vi "Input&output.vi"() -> ()   [LabVIEW 2021]
uses:
  Option control.ctl
panel:
  in  "Tab Control":enum32{"Page 2"}(tab)
  in  "LOG ID":string
  in  "OK":bool caption="OK2"
  in  "PASSWORD":string
  # "Enter opertor Name and ID\n and press OK"
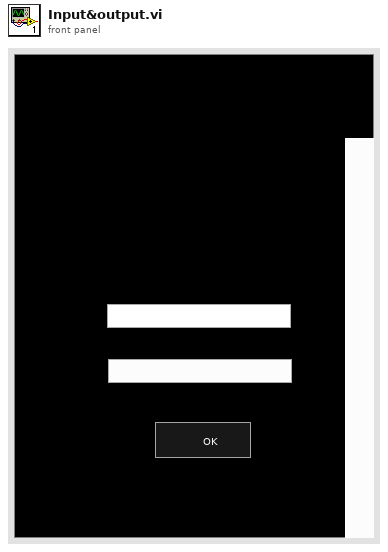
[diagram p1: front panel]
types:
  T1 = typedef "Option control.ctl" = enum16{"Input", "Output"}
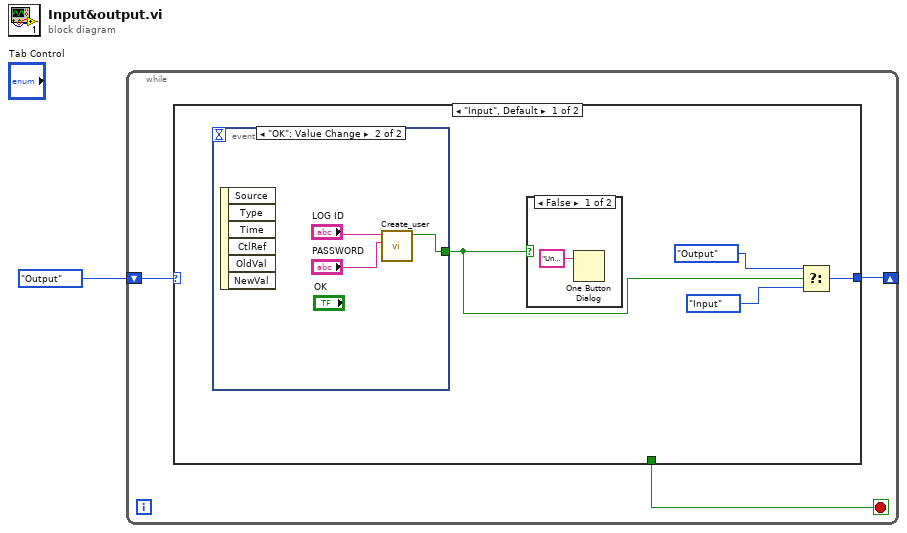
[diagram p0: block diagram]
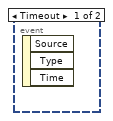
[diagram p3: hidden frame]
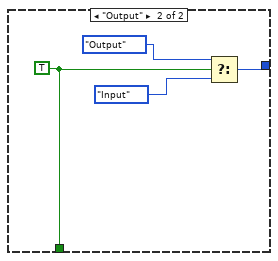
[diagram p4: hidden frame]
diagram:
  n1 = while {
    shift-right: [w3] -> _
    shift-left: Option_control."Output" -> [w4]
    stop <- w2 stop-if-true
    n2 = case shown="\"Input\", Default" w4 {
      tunnel: [w6 w14] -> w3
      tunnel: [_ w13] -> w2
      frame "Input", Default {
        n3 = event shown="[1] \"OK\": Value Change" {
          selector: _ -> [_ _]
          dyn-events: _ -> [_ _]
          timeout: _ -> [_ _]
          tunnel: [_ w10] -> w5
          event Timeout {
            n4 = event-data() -> ()  [unwired: 1 in, 3 out]
          }
          event "OK": Value Change {
            n5 = event-data() -> ()  [unwired: 1 in, 6 out]
            n6 = call "Create_user.vi"("Password"="PASSWORD", "Name"="LOG ID") -> ("Result"=w10:bool)  [unwired: 8 in, 1 out]
          }
        }
        n7 = case shown="False" w5 {
          frame False {
            n8 = One Button Dialog(message="Unable to Create a user") -> ()  [unwired: 1 in, 1 out]
          }
          frame True {
          }
        }
        n9 = Select(t=Option_control."Output", s=w5, f=Option_control."Input") -> (s? t:f=w6:T1)
      }
      frame "Output" {
        w13 = TRUE ("s")
        n10 = Select(t=Option_control."Output", s=w13, f=Option_control."Input") -> (s? t:f=w14:T1)
      }
    }
  }
